vi "Build VIHelpeks Project Example.vi"(4 "Open Build Log file":bool=TRUE, 5 "Show Progress Window":bool=TRUE, 6 "Open Help File":bool=TRUE, 7 "Apply help to the VI":bool, 8 "error in":errorcluster, 9 "Generate CHM File":bool, 10 "Generate new HHP File":bool, 11 "VIHelpeks Project File":path=path "Build VIHelpeks Project Example.hgprj") -> (0 "error out":errorcluster, 1 "Errors":i32, 2 "VI Help Info":T2(array[cluster]), 3 "Important Files":T3)   [LabVIEW 2014]
doc: "This example VI demonstrates the use of the VI Helpeks API for building help files. The VI processes a VI Helpeks project that is pre-configured to build help for this specific VI, meaning that the VI builds help for itself. By default, the VI creates an HTML help file and can optionally compile it into a CHM file. In addition, this example demonstrates how to configure and apply VI documentation properties using the toolkit's API VIs.\n\n<b>NOTICE:</b> In order to generate a CHM file, it is required to have Microsoft HTML Help Workshop installed on your computer."
uses:
  <vilib>/Platform/browser.llb/Open URL in Default Browser (path).vi
  vi.lib/addons/VI Helpeks/VIHelpeksAPI.lvlib
panel:
  in  "VI Help Linking":T1={"Help Targeting"=enum."relative", "Subfolder"="", "CHM Tag mode"=enum."HTML Filename"}
  # "This example VI demonstrates using of VI Helpeks API for building help files. The VI processes VI Helpeks project\nthat is preliminary configured to build help for this VI. This means that this VI builds help for itself. By default, the\nVI creates HTML help file and optionally can compile it to CHM file. In addition, this example demonstrates how to\nconfigure and apply VI help properties with the use of API VIs.\n\nIMPORTANT: It's strongly recommended to mass compile VI Helpeks before use it. If you haven't done this yet,\nmass compile it with the Tools>>VI Helpeks>>Mass compile VI Helpeks menu.\n\nIMPORTANT: Ensure VI Helpeks UI (Project Manager) is closed before starting this VI.\n\nIMPORTANT: Microsoft HTML Help Workshop must be installed on the computer in order to generate a CHM file.\nYou can download it for free at the Microsoft website:\nhttp://msdn.microsoft.com/en-us/library/ms669985.aspx"
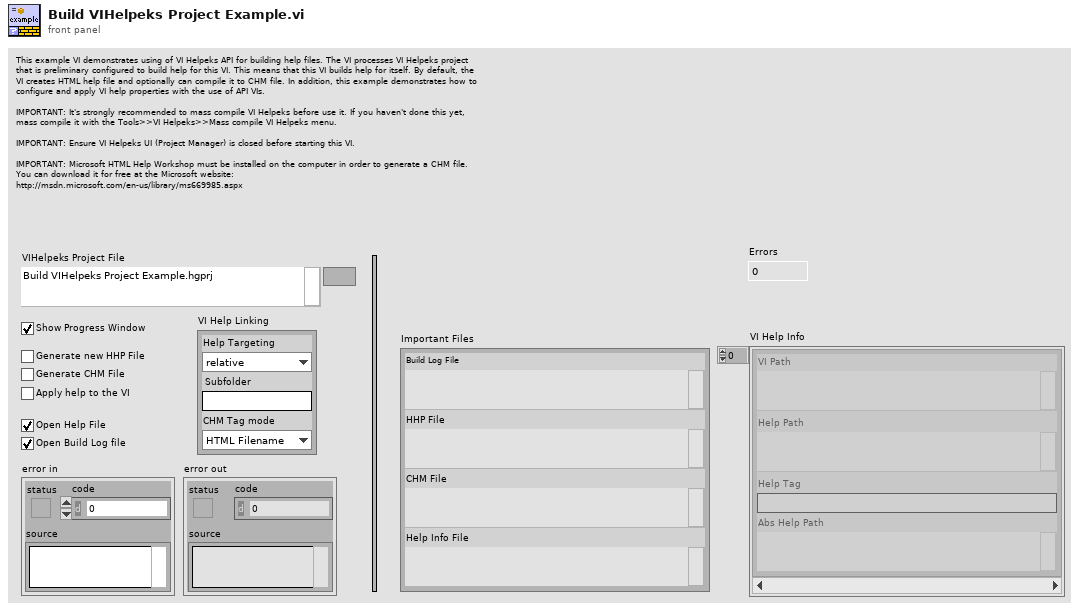
[diagram p1: front panel]
types:
  T1 = cluster{"Help Targeting":enum16{"absolute", "relative", "<helpdir>", "<userlib>", "<vilib>", "<instrlib>"}, "Subfolder":string, "CHM Tag mode":enum16{"HTML Filename", "Index Keyword"}}
  T2 = cluster{"VI Path":path, "Help Path":path, "Help Tag":string, "Abs Help Path":path}[]
  T3 = cluster{"Build Log File":path, "HHP File":path, "CHM File":path, "Help Info File":path}
  T4 = cluster{"Apply help to the VI":bool, "Apply help to the VI":bool}
  T5 = cluster{"Help Path":path, "Help Tag":string, "Abs Help Path":path}[]
  T6 = cluster{"Help Path":path, "Help Tag":string, "Abs Help Path":path}
  T7 = cluster{"Original File Path":path, "Help Path":path, "Help Tag":string, "Abs Help Path":path}
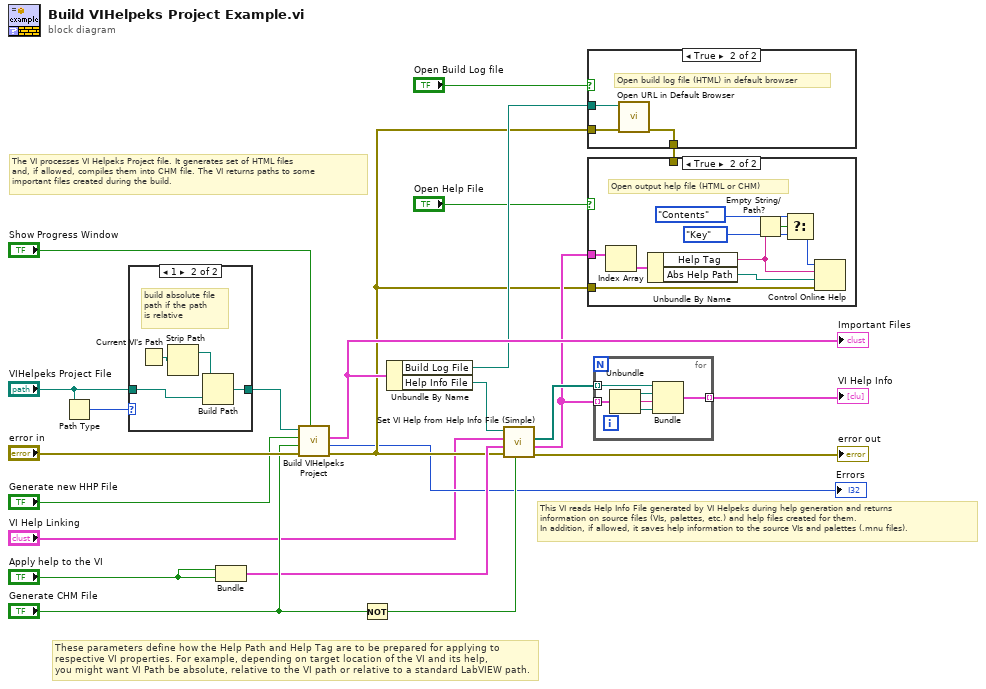
[diagram p0: block diagram]
diagram:
  # "These parameters define how the Help Path and Help Tag are to be prepared for applying to\nrespective VI properties. For example, depending on target location of the VI and its help,\nyou might want VI Path be absolute, relative to the VI path or relative to a standard LabVIEW path."
  # "The VI processes VI Helpeks Project file. It generates set of HTML files\nand, if allowed, compiles them into CHM file. The VI returns paths to some\nimportant files created during the build."
  # "This VI reads Help Info File generated by VI Helpeks during help generation and returns\ninformation on source files (VIs, palettes, etc.) and help files created for them.\nIn addition, if allowed, it saves help information to the source VIs and palettes (.mnu files)."
  n1 = Path Type(1:"VIHelpeks Project File") -> (0:w21:i16)
  n2 = case shown="1" w21 {
    tunnel: [w24 w25] -> w19
    tunnel: "VIHelpeks Project File" -> [w24 w26]
    frame Default {
    }
    frame 1 {
      # "build absolute file\npath if the path\nis relative"
      n3 = Current VI's Path() -> (path=w28:path)
      n4 = Strip Path(path=w28) -> (stripped path=w27:path)  [unwired: 1 out]
      n5 = Build Path(base path=w27, name or relative path=w26) -> (appended path=w25:path)
    }
  }
  n6 = Bundle("Apply help to the VI"="Apply help to the VI", "Apply help to the VI"="Apply help to the VI") -> (w12:T4)  [unwired: 1 in]
  n7 = call "Build VIHelpeks Project.vi"("Show Progress Window (T)"="Show Progress Window", "error in"="error in", "Generate CHM (T)"="Generate CHM File", "Generate HHP (T)"="Generate new HHP File", "VIHelpeks Project File"=w19) -> ("error out"=w5:errorcluster, "Errors"=→"Errors":i32, "Paths"=w22:T3)  [unwired: 3 in, 1 out]
  "Important Files" <- w22
  n8 = Not(x="Generate CHM File") -> (.not. x?=w17:bool)
  n9 = Unbundle By Name(w22) -> ("Build Log File"=w11:path, "Help Info File"=w18:path)
  n10 = call "Set VI Help from Help Info File (Simple).vi"("Link to HTML (F)"=w17, "error in"=w5, "Save Params"=w12, "Build Params"="VI Help Linking", "Help Info File"=w18) -> ("error out"=→"error out":errorcluster, "Source Files Help Info"=w9:T5, "Source File Paths"=w15:path[])  [unwired: 3 in, 1 out]
  n11 = case shown="True" "Open Build Log file" {
    tunnel: w11 -> [_ w31]
    tunnel: w5 -> [_ w30]
    tunnel: [_ w29] -> w3
    frame False {
    }
    frame True {
      # "Open build log file (HTML) in default browser"
      n12 = call-poly <vilib>:"Open URL in Default Browser.vi"("error in (no error)"=w30, "path"=w31) -> ("error out"=w29:errorcluster)  [unwired: 4 in, 1 out]
    }
  }
  n13 = case shown="True" "Open Help File" {
    tunnel: w9 -> [_ w40]
    tunnel: w5 -> [_ w32]
    tunnel: w3 -> [_ _]
    frame False {
    }
    frame True {
      # "Open output help file (HTML or CHM)"
      n14 = Index Array(array=w40) -> (element=w39:T6)  [unwired: 1 in]
      n15 = Unbundle By Name(w39) -> ("Help Tag"=w36:string, "Abs Help Path"=w38:path)
      n16 = Empty String/Path?(string/path=w36) -> (empty?=w37:bool)
      n17 = Select(t=enum16{"Contents", "Key", "Close"}."Contents" ("Operation"), s=w37, f=enum16{"Contents", "Key", "Close"}."Key" ("Operation")) -> (s? t:f=w35:enum16{"Contents", "Key", "Close"})
      n18 = Control Online Help(1:w32, 2:w38, 3:w36, 4:w35) -> ()  [unwired: 1 out]
    }
  }
  n19 = for {
    tunnel: w9 -> [w46] mode=indexing
    tunnel: w15 -> [w45] mode=indexing
    tunnel: [w42] -> w14 mode=indexing
    n20 = Unbundle(w46) -> ("Help Path"=w44:path, "Help Tag"=w43:string, "Abs Help Path"=w41:path)
    n21 = Bundle("Original File Path"=w45, "Help Path"=w44, "Help Tag"=w43, "Abs Help Path"=w41) -> (w42:T7)  [unwired: 1 in]
  }
  "VI Help Info" <- w14
